vi "Create Group from Config.vi"(7 "Group Type (Abstract)":refnum<class "Group.lvclass">, 8 "error in (no error)":errorcluster, 10 "Group Config":refnum<class "Group Config.lvclass">, 11 "Module in":refnum<class "Module.lvclass">) -> (0 "error out":errorcluster, 2 "Group":refnum<class "Group.lvclass">, 3 "Module out":refnum<class "Module.lvclass">)   [LabVIEW 2020, in "Volatus.lvlib" / "Module.lvclass"]
uses:
  Module.lvclass
  VolatusConfig/Group/Group Config.lvclass
  C:/dev/lv20CE/relink/lv-volatus/VolatusConfig/VolatusConfigElement/VolatusConfigElement.lvclass
  lv-vecto/Vecto/Group/Group.lvclass
  VolatusConfig/VolatusConfigElement/VolatusConfigElement.lvclass/VolatusConfigElement.ctl
  lv-vecto/Vecto/Group DBL/Group DBL.lvclass
  C:/dev/lv20CE/relink/lv-vecto/Vecto/Group/Group.lvclass
  lv-vecto/Vecto/Group STR/Group STR.lvclass
  lv-vecto/Vecto/Group BOOL/Group BOOL.lvclass
  VolatusConfig/VolatusConfigElement/Element.vi
  VolatusConfig/VolatusConfigElement/Lookup Child by Name.vi
  VolatusConfig/Channel/Channel Config.lvclass
  lv-cdm/CDM-Config/Config Element/Lookup Child by Name.vi
  lv-cdm/CDM-Config/Config Element/Value (String).vi
  Module.lvclass/Module.ctl
  VolatusConfig/VolatusConfigElement/VolatusConfigElement.lvclass
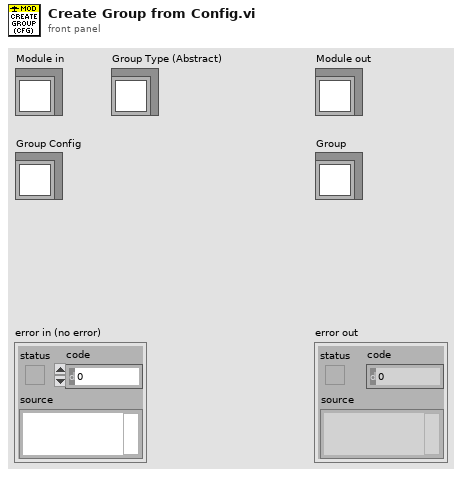
[diagram p1: front panel]
types:
  T1 = typedef "VectoConfig.lvlib/Group Data Type.ctl" = enum16{"Double", "String", "Bool"}
  T2 = typedef "VectoConfig.lvlib/Endpoint.ctl" = cluster{"Address":string, "Port":u16}
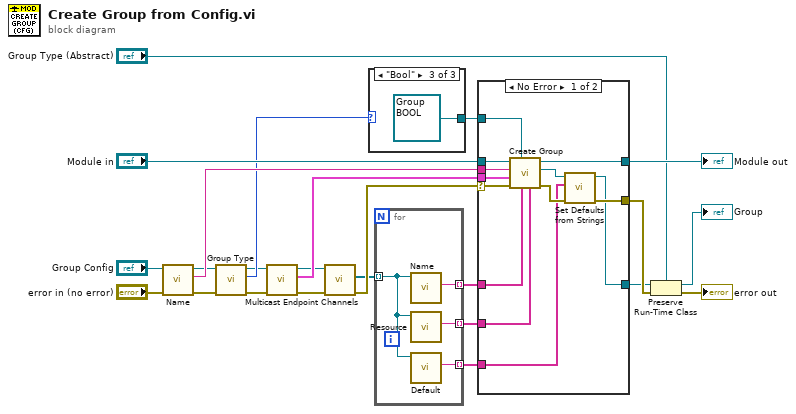
[diagram p0: block diagram]
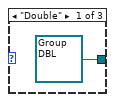
[diagram p2: hidden frame]
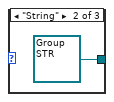
[diagram p3: hidden frame]
diagram:
  n1 = call "Name.vi"("error in (no error)"="error in (no error)", "VolatusConfigElement in"="Group Config") -> ("error out"=w10:errorcluster, "Name"=w18:string, "VolatusConfigElement out"=w17:refnum<class "Group Config.lvclass">)  [unwired: 7 in]
  n2 = call "Group Type.vi"("error in (no error)"=w10, "Group in"=w17) -> ("error out"=w9:errorcluster, "Group Data Type"=w16:T1, "Group out"=w14:refnum<class "Group Config.lvclass">)  [unwired: 7 in]
  n3 = call "Multicast Endpoint.vi"("error in (no error)"=w9, "Group in"=w14) -> ("error out"=w8:errorcluster, "Multicast Endpoint"=w13:T2, "Group out"=w12:refnum<class "Group Config.lvclass">)  [unwired: 7 in]
  n4 = call "Channels.vi"("error in (no error)"=w8, "Group in"=w12) -> ("error out"=w22:errorcluster, "Channels"=w7:refnum<class "Channel Config.lvclass">[])  [unwired: 7 in, 1 out]
  n5 = case shown="\"Bool\"" w16 {
    tunnel: [refnum<class "Group DBL.lvclass"> refnum ("Vecto.lvlib:Group.lvclass") refnum<class "Group STR.lvclass"> refnum ("Vecto.lvlib:StringGroup.lvclass") refnum<class "Group BOOL.lvclass"> refnum ("Vecto.lvlib:StringGroup.lvclass")] -> w15
    frame "Double" {
    }
    frame "String" {
    }
    frame "Bool" {
    }
  }
  n6 = for {
    tunnel: w7 -> [w28] mode=indexing
    tunnel: [w31] -> w6 mode=indexing
    tunnel: [w30] -> w5 mode=indexing
    tunnel: [w29] -> w1 mode=indexing
    n7 = call "Name.vi"("VolatusConfigElement in"=w28) -> ("Name"=w30:string)  [unwired: 8 in, 2 out]
    n8 = call "Resource.vi"("Channel in"=w28) -> ("Resource"=w31:string)  [unwired: 8 in, 2 out]
    n9 = call "Default.vi"("Channel in"=w28) -> ("Default"=w29:string)  [unwired: 8 in, 2 out]
  }
  n10 = case shown="No Error" w22 {
    selector: w22 -> [w43 w45]
    tunnel: [w33 w45] -> w24
    tunnel: "Module in" -> [w42 w46]
    tunnel: [w41 w46] -> w20
    tunnel: w18 -> [w40 _]
    tunnel: w15 -> [w39 _]
    tunnel: w13 -> [w38 _]
    tunnel: w6 -> [w37 _]
    tunnel: w5 -> [w36 _]
    tunnel: [w32 _] -> w4
    tunnel: w1 -> [w34 _]
    frame No Error {
      n11 = call "Create Group.vi"("Channel Resources (Unset)"=w37, "Channel Names"=w36, "Group Type"=w39, "error in (no error)"=w43, "Multicast Config (Local Only)"=w38, "Group Name"=w40, "Module in"=w42) -> ("error out"=w44:errorcluster, "Group"=w35:refnum<class "Group.lvclass">, "Module out"=w41:refnum<class "Module.lvclass">)  [unwired: 2 in]
      n12 = call-dynamic "Set Defaults from Strings.vi"("error in (no error)"=w44, "Default Strings"=w34, "Group in"=w35) -> ("error out"=w33:errorcluster, "Group out"=w32:refnum<class "Group.lvclass">)  [unwired: 7 in]
    }
    frame Error {
    }
  }
  "Module out" <- w20
  n13 = Preserve Run-Time Class(object in=w4, error in=w24, 2:"Group Type (Abstract)") -> (object out=→"Group":refnum<class "Group.lvclass">, error out=→"error out":errorcluster)
